vi "W32B Create CLFN.vi"(0 "VI reference":refnum<vi>, 1 "run in UI thread?":bool, 5 "function name":string, 7 "library path":path, 9 "parameter info":T1(array[cluster]), 11 "error in":errorcluster) -> (4 "CLFN terminals":refnum<vi>[](array[refnum]), 15 "error out":errorcluster)   [LabVIEW 2020]
doc: "Places a Call Library Function Node on the block diagram of the VI behind VI reference and configures it by VI Server: library path, function name, the calling convention (stdcall/WINAPI for a DLL, C for the library LabVIEW - the functions LabVIEW itself exports), the thread it runs in (any thread, or LabVIEW's UI thread when run in UI thread? is TRUE), and parameter info (element 0 is the return value). Returns the node's terminals in LabVIEW's order: 0 path in, 1 path out, 2 error in, 3 error out, 4/5 return value, then an input/output pair per parameter."
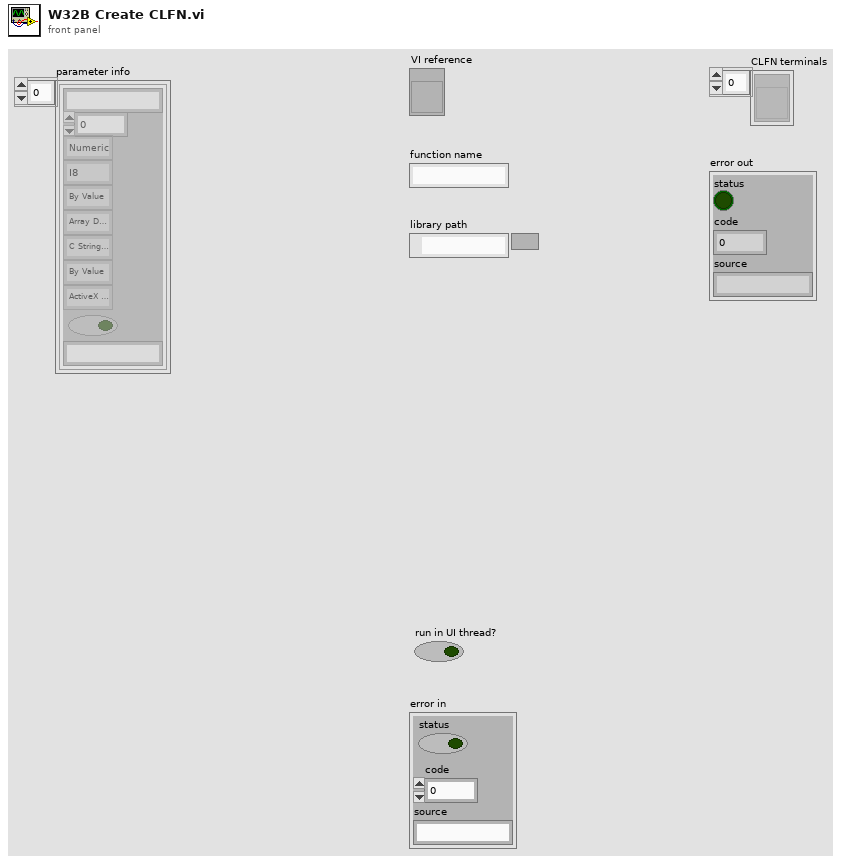
[diagram p1: front panel]
types:
  T1 = cluster{"Parameter Name":string, "Num Dimensions":i32, "Parameter Type":enum16{"Numeric", "Array", "String", "Waveform", "Digital Waveform", "Digital Table", "ActiveX", "Any", "Instance Data Pointer", "Void"}, "Numeric Type":enum16{"I8", "I16", "I32", "I64", "U8", "U16", "U32", "U64", "SGL", "DBL", "PTR INT", "PTR UINT"}, "Param Passing":enum16{"By Value", "Pointer To Value"}, "Array Passing":enum16{"Array Data Pointer", "Array Handle", "Array Handle Pointer"}, "String Passing":enum16{"C String Pointer", "Pascal String Pointer", "String Handle", "String Handle Pointer"}, "Adapt Format":enum16{"By Value", "Pointer To Value"}, "ActiveX Types":enum16{"ActiveX Variant Pointer", "IDispatch* Pointer", "IUnknown* Pointer"}, "Const (unused)":bool, "Minimum Size":string}[]
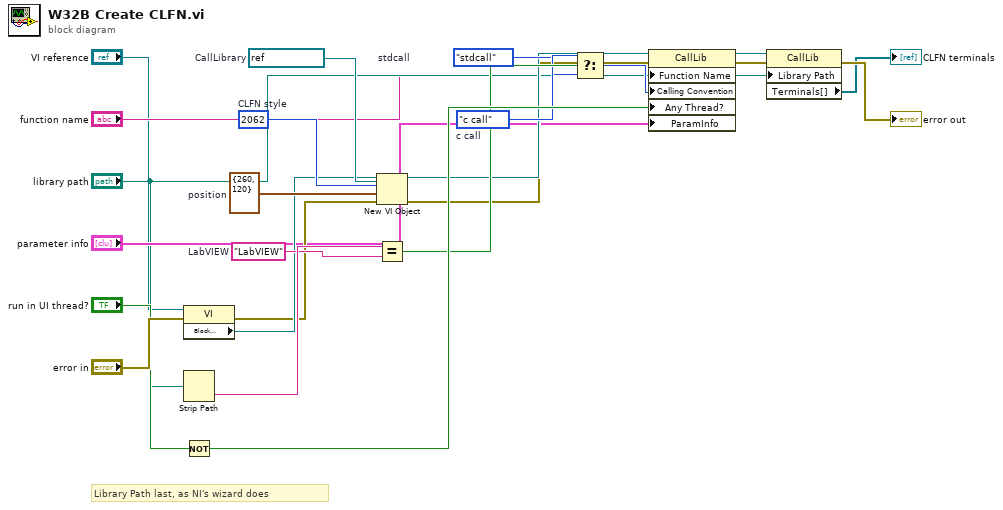
[diagram p0: block diagram]
diagram:
  w18 = "LabVIEW"  # LabVIEW
  w17 = enum32{"c call", "stdcall"}."c call"  # c call
  w16 = enum32{"c call", "stdcall"}."stdcall"  # stdcall
  w13 = cluster{"Horizontal":i16, "Vertical":i16} {"Horizontal"=260, "Vertical"=120}  # position
  w12 = 2062  # CLFN style
  w11 = refnum<vi> refnum  # CallLibrary
  # "Library Path last, as NI's wizard does"
  n1 = property class="VI"(reference="VI reference", error in="error in") -> (error out=w9:errorcluster, "Block Diagram"=w10:refnum<vi>)  [unwired: 1 out]
  n2 = Strip Path(path="library path") -> (name=w19:string)  [unwired: 1 out]
  n3 = Not(x="run in UI thread?") -> (.not. x?=w22:bool)
  n4 = New VI Object(vi object class=w11, owner refnum=w10, style=w12, position/next to=w13, 8:w9) -> (object refnum=w15:refnum<vi>, 0:w14:errorcluster)  [unwired: 3 in]
  n5 = Equal?(x=w19, y=w18) -> (x = y?=w20:bool)
  n6 = Select(t=w17, s=w20, f=w16) -> (s? t:f=w21:enum32{"c call", "stdcall"})
  n7 = property class="CallLib"(reference=w15, error in=w14, "Function Name"="function name", "Calling Convention"=w21, "Any Thread?"=w22, "ParamInfo"="parameter info") -> (reference out=w23:refnum<vi>, error out=w24:errorcluster)
  n8 = property class="CallLib"(reference=w23, error in=w24, "Library Path"="library path") -> (error out=→"error out":errorcluster, "Terminals[]"=→"CLFN terminals":refnum<vi>[])  [unwired: 1 out]
